vi "Measurement UI.vi"() -> ()   [LabVIEW 2023, in "FPT Intermodulation UI.lvlib"]
uses:
  FPT Intermodulation UI.lvlib
panel:
  in  "Measurement Graph":T1(tab)
  out "Graph Combined":T2(graph)
  out "Graph DUT Gain":T2(graph)
  out "Graph Intermodulation":T2(graph)
  out "Graph TOI":T2(graph)
  out "Graph Fundamental":T2(graph)
  in  "Power sequencing file validity check":bool
  out "TS_Intermodulation Slope (dBm)":dbl[][](array[numeric])
  out "TS_Fundamental Slope (dBm)":dbl[][](array[numeric])
  out "Final Target Pout (dBm)":dbl
  out "All Data":dbl[][](array[numeric])
  out "TS_DUT Gain (dBm)":dbl[][](array[numeric])
  out "TS_TOI (dBm)":dbl[][](array[numeric])
  out "TS_IMD (dBm)":dbl[][](array[numeric])
  out "TS_Fundamental (dBm)":dbl[][](array[numeric])
  out "Typical OIP3 (dBm)":dbl
  out "x-axis label":string
  in  "Power sequencing file path":string
  in  "RFSG name":string="5842_0"
  in  "RFSG attenuation mode":T3(ring)=enum."Constant Attenuation"
  in  "RFSG s2p file path":string
  in  "RFmx name":string="5842_0"
  in  "RFmx attenuation mode":T3(ring)=enum."Constant Attenuation"
  in  "RFmx s2p file path":string
  out "All Graph Reference":refnum<vi>[](array[refnum])
  out "All Plots Data":T4(array[cluster])
  in  "IM_Sweep Mode":enum32{"Power", "Frequency", "Tone Spacing"}(ring) caption="Sweep Mode"
  out "MeasTable_Fix":string[][](table)
  out "MeasTable":string[][](table)
  in  "Tab Control":T5(tab)
  in  "Power sequencing file path_update":path caption="Power Sequencing File Path"
  in  "RFSG name_update":refnum<k15> caption="RFSG Name"
  in  "RFSG attenuation mode_tab":T3(tab)=enum."s2p File" caption="RFSG Attenuation Mode"
  in  "RFSG external attenuation (dB)":dbl caption="External Attenuation" format="%#.3pdB"
  in  "RFSG s2p file path_update":path caption="S2P File Path"
  in  "RFSG s-parameters orientation":enum32{"Port1 Towards DUT", "Port2 Towards DUT"}(ring) caption="Orientation"
  in  "RFmx name_update":refnum<k15> caption="RFmx Name"
  in  "RFmx attenuation mode_tab":T3(tab) caption="RFmx Attenuation Mode"
  in  "RFmx external attenuation (dB)":dbl caption="External Attenuation" format="%#.3pdB"
  in  "RFmx s2p file path_update":path caption="S2P File Path"
  in  "RFmx s-parameters orientation":enum32{"Port1 Towards DUT", "Port2 Towards DUT"}(ring) caption="Orientation"
  in  "RFSG port":string(combo)="port1" caption="RFSG Port"
  in  "RFmx port":string(combo)="port2" caption="RFmx Port"
  in  "RFmx Reference Level (dBm)":dbl=10.0 caption="Reference Level" format="%#.3fdBm"
  in  "RFSG Generation IQ Rate (S/s)":dbl=1250000000.0 caption="Generation IQ Rate" format="%#.3pS/s"
  in  "Start Pin Per Tone (dBm)":dbl=-20.0 caption="Start Pin Per Tone" format="%#.3fdBm"
  in  "Start Center Frequency (Hz)":dbl=8000000000.0 caption="Start Center Frequency" format="%#.3pHz"
  in  "Start Tone Spacing (Hz)":dbl=1000000.0 caption="Start Tone Spacing" format="%#.3pHz"
  in  "Sweep Delay (ms)":u32 format="%#.3pms"
  in  "Sweep Mode_tab":enum32{"Power", "Frequency", "Tone Spacing"}(tab)=enum."Tone Spacing" caption="Sweep Mode"
  in  "Power Sweep End":dbl format="%#.fdBm"
  in  "Power Sweep Step":dbl=1.0 format="%#.fdB"
  in  "Target Pout Per Tone (dBm)":dbl caption="Target Pout Per Tone" format="%#.3fdBm"
  in  "Frequency Sweep End":dbl=12000000000.0 format="%#.pHz"
  in  "Frequency Sweep Step":dbl=100000000.0 format="%#.pHz"
  in  "Tone Spacing Sweep End":dbl=10000000.0 format="%#.pHz"
  in  "Tone Spacing Sweep Step":dbl=1000000.0 format="%#.pHz"
  in  "Mode of operation":T6(ring) caption="Configuration"
  out "Status":string
  # "Intermodulation"
  # "Sweep Options"
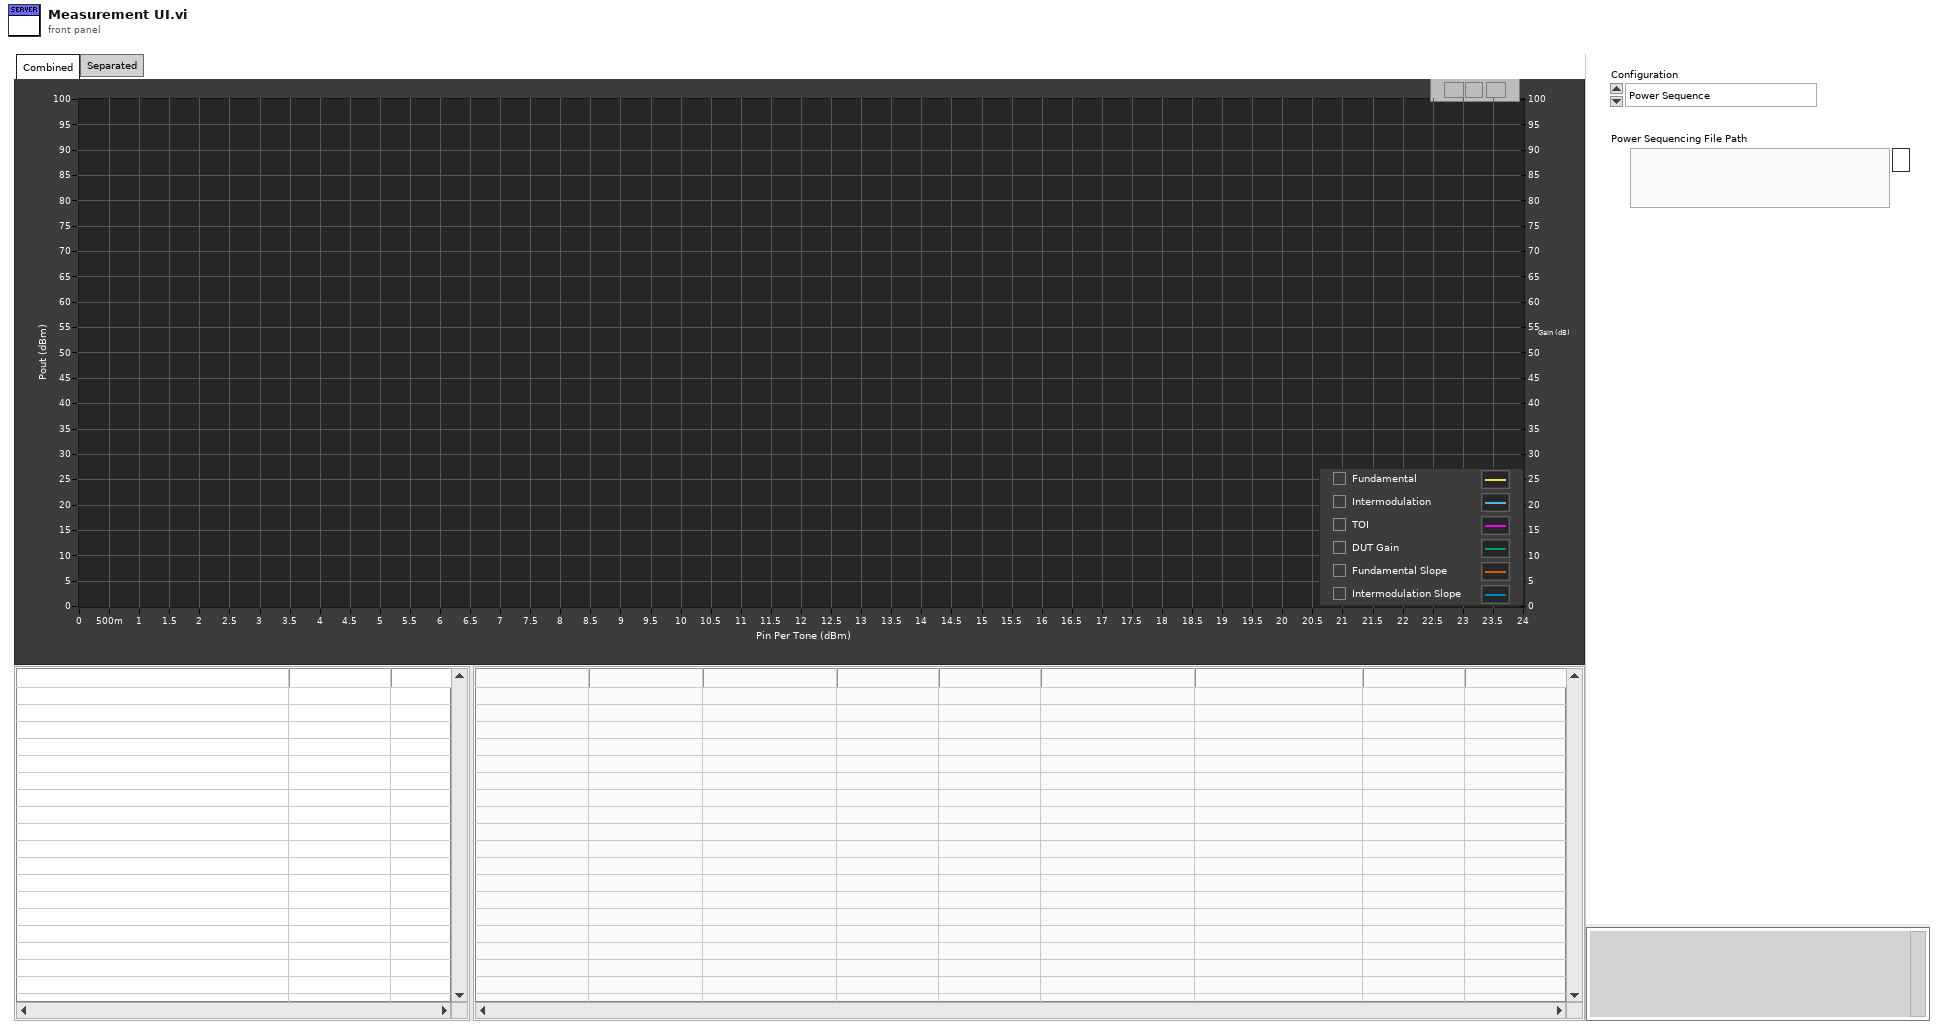
[diagram p1: front panel]
types:
  T1 = enum32{"Combined", "Separated", "Hidden Controls"}
  T2 = cluster{"Load currents":dbl[], "Efficiency":dbl[]}[]
  T3 = enum32{"<None>", "Constant Attenuation", "s2p File"}
  T4 = cluster{"X-axis values":dbl[], "Y-axis values":dbl[]}[]
  T5 = enum32{"Power Sequence", "Correction", "Measurement 1"}
  T6 = enum32{"Power Sequence", "HW + Correction", "Measurement 1"}
  T7 = enum8{"Enabled", "Disabled", "Disabled and Grayed Out"}
  T8 = cluster{"Shift":bool, "Ctrl":bool, "Alt":bool, "Cmd":bool, "Opt":bool}
  T9 = cluster{"TS_Fundamental Slope (dBm)":dbl[], "TS_Fundamental Slope (dBm)":dbl[]}
  T10 = cluster{"TS_Fundamental Slope (dBm)":dbl[], "TS_Intermodulation Slope (dBm)":dbl[]}
  T11 = cluster{"TS_Fundamental Slope (dBm)":dbl[], "TS_Intermodulation Slope (dBm)":dbl[]}[]
  T12 = cluster{"TS_Fundamental (dBm)":dbl[], "TS_Fundamental (dBm)":dbl[]}
  T13 = cluster{"TS_Fundamental (dBm)":dbl[], "TS_IMD (dBm)":dbl[]}
  T14 = cluster{"TS_Fundamental (dBm)":dbl[], "TS_TOI (dBm)":dbl[]}
  T15 = cluster{"TS_Fundamental (dBm)":dbl[], "TS_DUT Gain (dBm)":dbl[]}
  T16 = cluster{"X-axis values":dbl[], "Y-axis values":dbl[]}
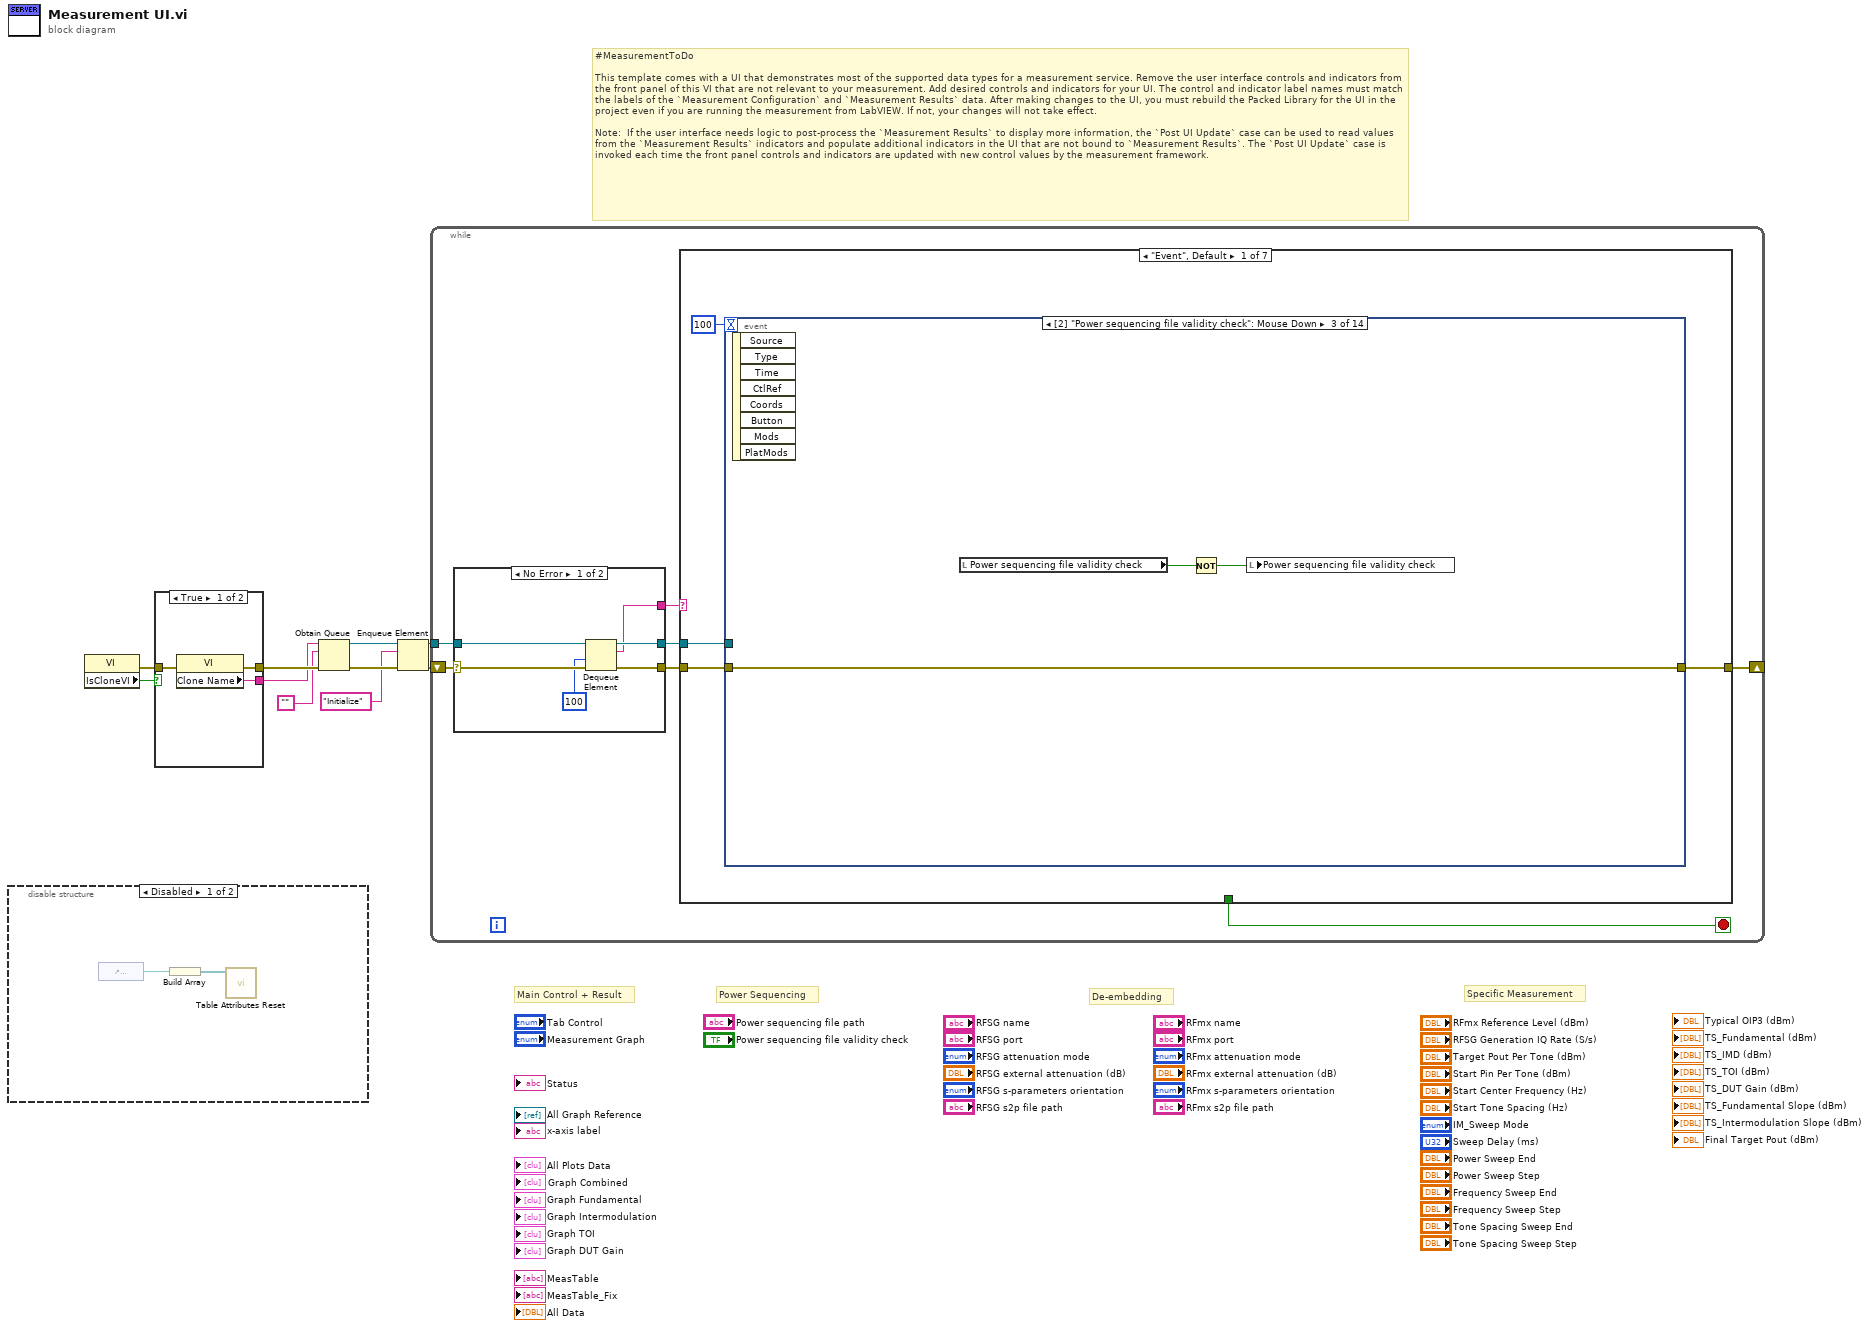
[diagram p0: block diagram]
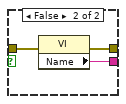
[diagram p3: hidden frame]
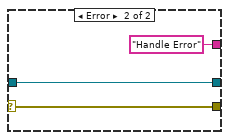
[diagram p4: hidden frame]
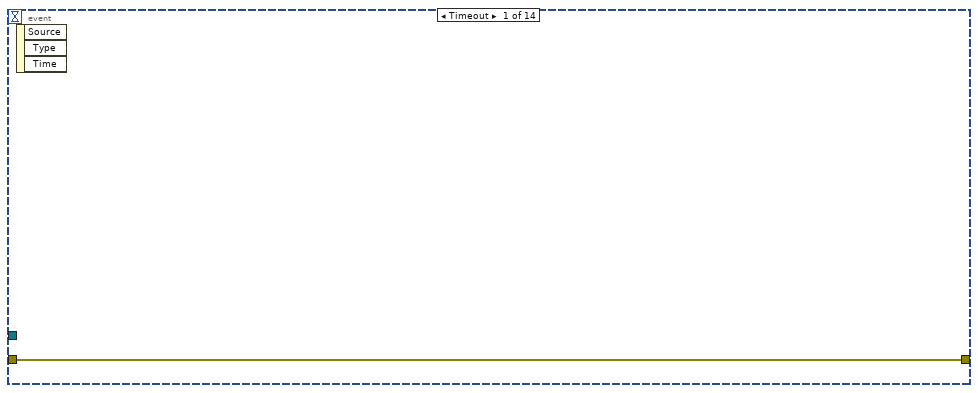
[diagram p5: hidden frame]
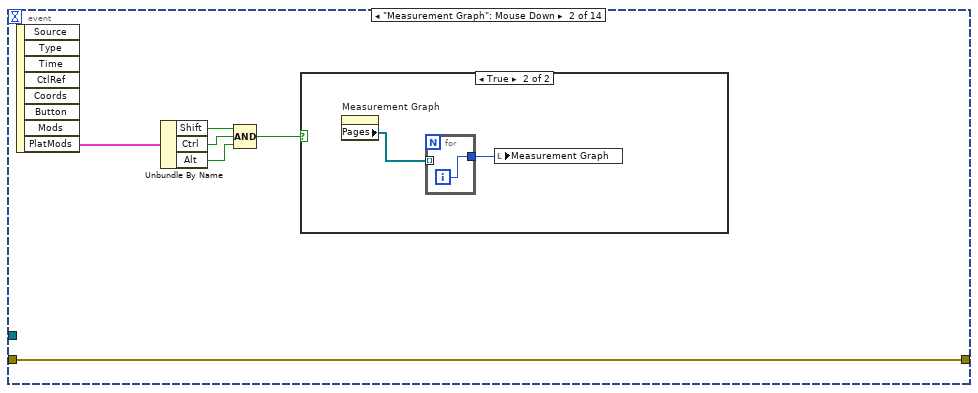
[diagram p6: hidden frame]
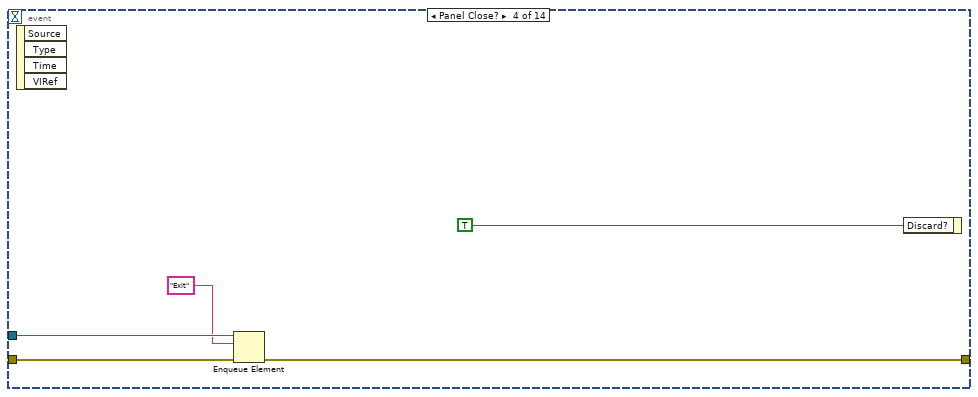
[diagram p8: hidden frame]
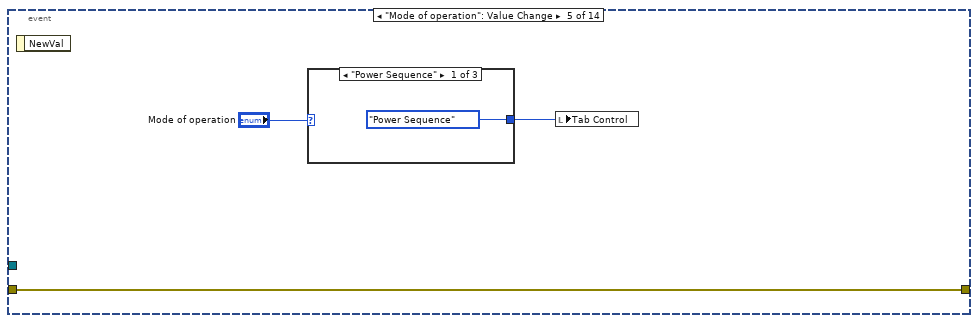
[diagram p9: hidden frame]
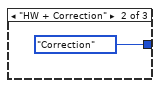
[diagram p10: hidden frame]
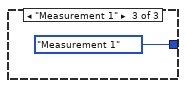
[diagram p11: hidden frame]
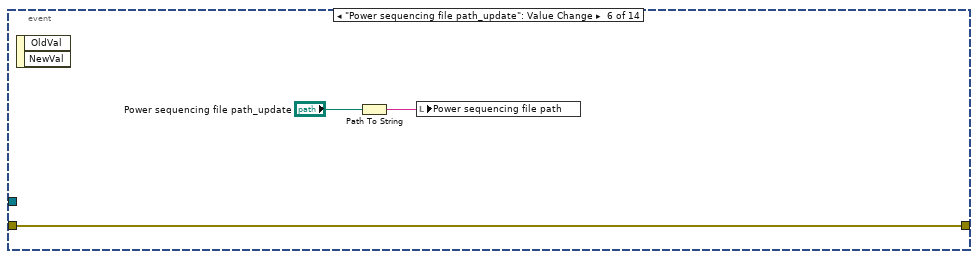
[diagram p12: hidden frame]
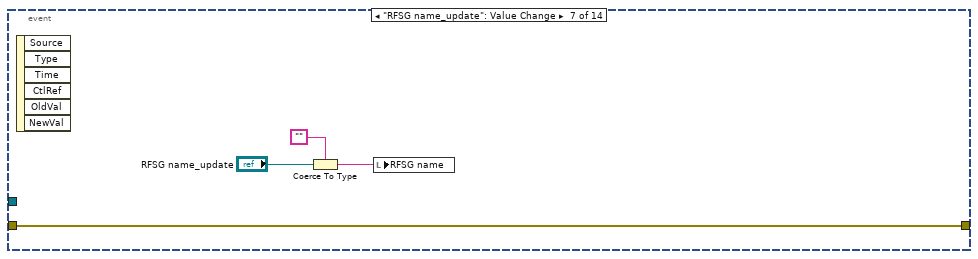
[diagram p13: hidden frame]
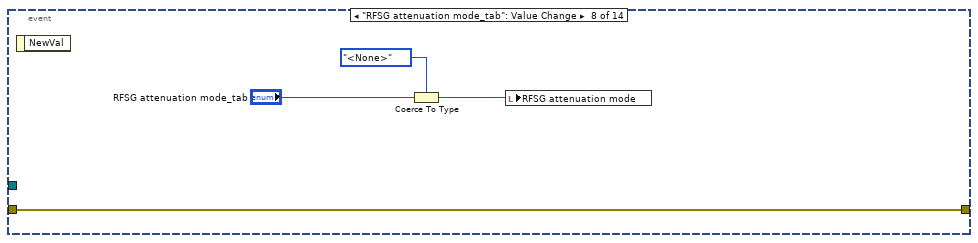
[diagram p14: hidden frame]
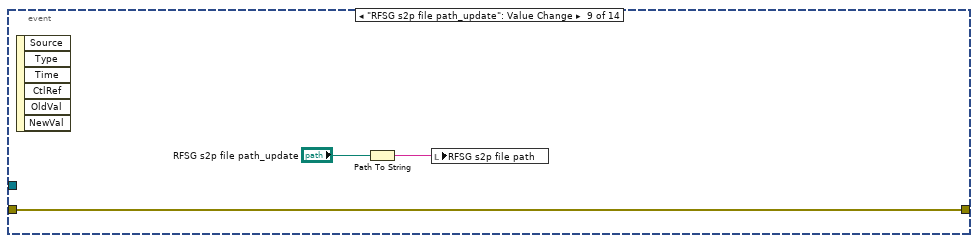
[diagram p15: hidden frame]
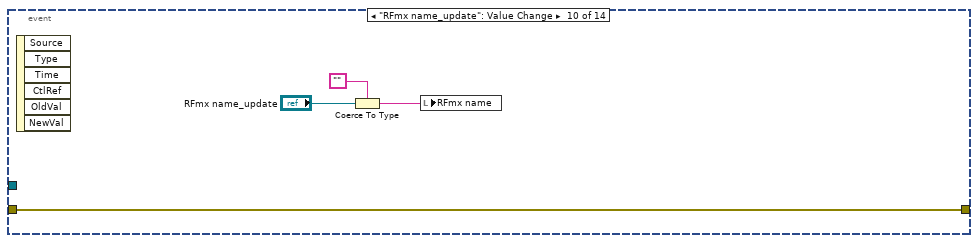
[diagram p16: hidden frame]
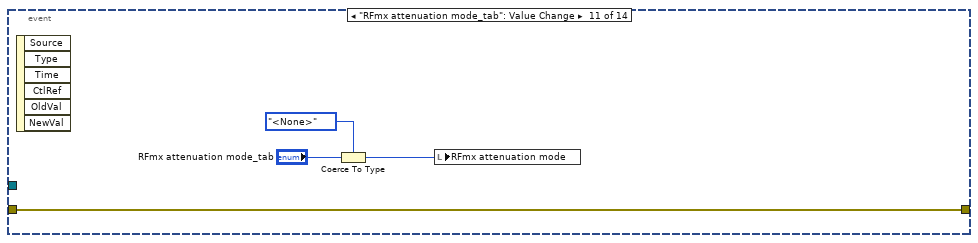
[diagram p17: hidden frame]
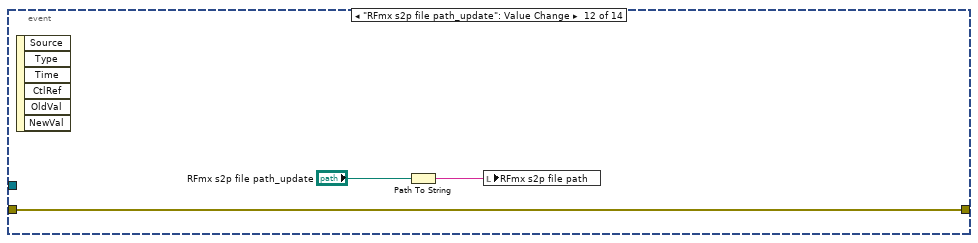
[diagram p18: hidden frame]
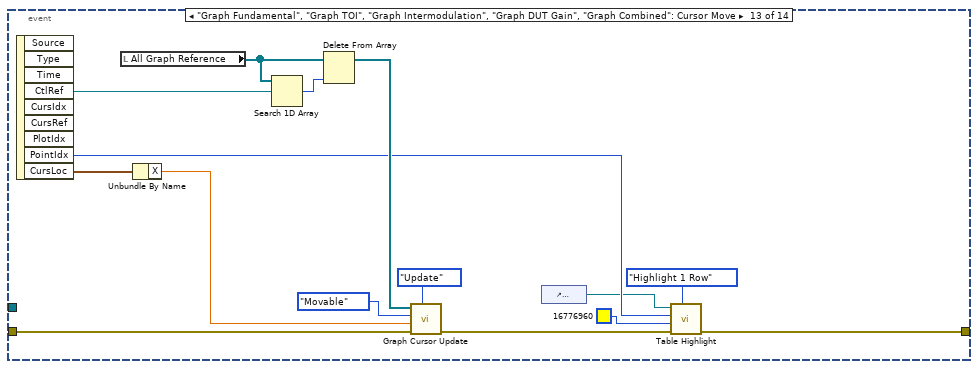
[diagram p19: hidden frame]
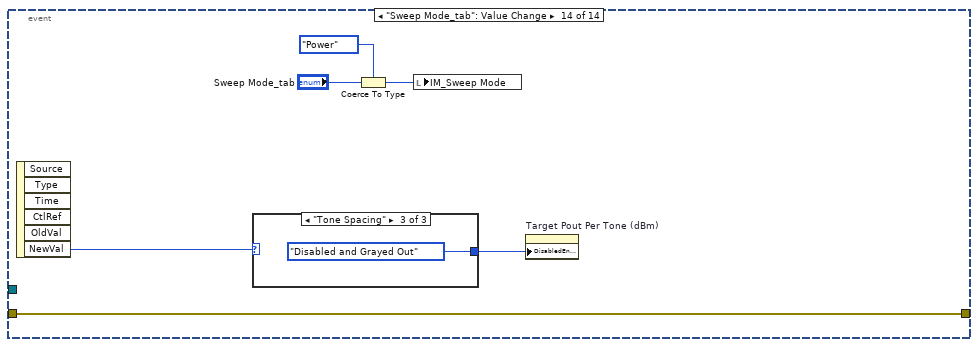
[diagram p20: hidden frame]
diagram:
  # "Specific Measurement"
  # "De-embedding"
  # "Power Sequencing"
  # "Main Control + Result"
  # "#MeasurementToDo  \n\nThis template comes with a UI that demonstrates most of the supported data types for a measurement service. Remove the user interface controls and indicators from the front panel of this VI that are not relevant to your measurement. Add desired controls and indicators for your UI. The control and indicator label names must match the labels of the `Measurement Configuration` and `Measurement Results` data. After making changes to the UI, you must rebuild the Packed Library for the UI in the project even if you are running the measurement from LabVIEW. If not, your changes will not take effect.\n\nNote:  If the user interface needs logic to post-process the `Measurement Results` to display more information, the `Post UI Update` case can be used to read values from the `Measurement Results` indicators and populate additional indicators in the UI that are not bound to `Measurement Results`. The `Post UI Update` case is invoked each time the front panel controls and indicators are updated with new control values by the measurement framework."
  n1 = disable-structure shown="Disabled" {
    frame Disabled {
      n2 = control-ref of="MeasTable"() -> (w12:refnum<vi>)
      n3 = Build Array(w12) -> (w11:refnum<vi>[])
      n4 = call "Table Attributes Reset.vi"("Table Refs"=w11) -> ()  [unwired: 11 in]
    }
    frame Enabled {
    }
  }
  n5 = property class="VI"() -> (error out=w1:errorcluster, "IsCloneVI"=w2:bool)  [unwired: 2 in, 1 out]
  n6 = case shown="True" w2 {
    tunnel: [w15 w18] -> w10
    tunnel: [w14 w17] -> w9
    tunnel: w1 -> [w13 w16]
    frame True {
      n7 = property class="VI"(error in=w13) -> (error out=w15:errorcluster, "Clone Name"=w14:string)  [unwired: 1 in, 1 out]
    }
    frame False {
      n8 = property class="VI"(error in=w16) -> (error out=w18:errorcluster, "Name"=w17:string)  [unwired: 1 in, 1 out]
    }
  }
  n9 = Obtain Queue(name (unnamed)=w9, element data type="", error in (no error)=w10) -> (queue out=w6:refnum<queue>, error out=w8:errorcluster)  [unwired: 2 in, 1 out]
  n10 = Enqueue Element(queue=w6, element="Initialize", error in (no error)=w8) -> (queue out=w5:refnum<queue>, error out=w7:errorcluster)  [unwired: 1 in, 1 out]
  n11 = while {
    shift-right: [w20] -> _
    shift-left: w7 -> [w25]
    tunnel: w5 -> [w23]
    stop <- w19 stop-if-true
    n12 = case shown="No Error" w25 {
      selector: w25 -> [w31 w34]
      tunnel: [w30 w34] -> w24
      tunnel: w23 -> [w29 w33]
      tunnel: [w28 w33] -> w22
      tunnel: [w27 "Handle Error"] -> w21
      frame No Error {
        n13 = Dequeue Element(queue=w29, timeout in ms (-1)=100, error in (no error)=w31) -> (queue out=w28:refnum<queue>, element=w27:string, error out=w30:errorcluster)  [unwired: 1 out]
      }
      frame Error {
      }
    }
    n14 = case shown="\"Event\", Default" w21 {
      tunnel: w24 -> [w37 w123 w175 w216 w240 w254 w255]
      tunnel: w22 -> [w35 _ w174 w215 _ w252 _]
      tunnel: [w38 w123 w175 w205 w240 w249 w255] -> w20
      tunnel: [_ _ _ _ _ TRUE _] -> w19
      frame "Event", Default {
        n15 = event shown="[2] \"Power sequencing file validity check\": Mouse Down" {
          selector: _ -> [_ _ _ _ _ _ _ _ _ _ _ _ _ _]
          dyn-events: _ -> [_ _ _ _ _ _ _ _ _ _ _ _ _ _]
          timeout: 100 -> [_ _ _ _ _ _ _ _ _ _ _ _ _ _]
          tunnel: [w39 w45 w51 w54 w58 w63 w66 w72 w74 w77 w83 w85 w92 w108] -> w38
          tunnel: w37 -> [w39 w45 w51 w55 w58 w63 w66 w72 w74 w77 w83 w85 w102 w108]
          tunnel: w35 -> [_ _ _ w53 _ _ _ _ _ _ _ _ _ _]
          event Timeout {
            n16 = event-data() -> ()  [unwired: 1 in, 3 out]
          }
          event "Measurement Graph": Mouse Down {
            n17 = event-data() -> ("PlatMods"=w44:T8)  [unwired: 1 in, 7 out]
            n18 = Unbundle By Name(w44) -> ("Shift"=w43:bool, "Ctrl"=w42:bool, "Alt"=w41:bool)
            n19 = Compound Arithmetic op=AND(w43, w42, w41) -> (w40:bool)
            n20 = case shown="True" w40 {
              frame False {
              }
              frame True {
                n21 = property on="Measurement Graph" class="TabCtl (strict)"() -> ("Pages"=w47:refnum<vi>[])  [unwired: 2 in, 2 out]
                n22 = for {
                  tunnel: w47 -> [_] mode=indexing
                  tunnel: [w48] -> w46
                  i -> [w48]
                }
                n23 = local write "Measurement Graph"(w46) -> ()
              }
            }
          }
          event "Power sequencing file validity check": Mouse Down {
            n24 = event-data() -> ()  [unwired: 1 in, 8 out]
            n25 = local read "Power sequencing file validity check"() -> (w50:bool)
            n26 = Not(x=w50) -> (.not. x?=w49:bool)
            n27 = local write "Power sequencing file validity check"(w49) -> ()
          }
          event Panel Close? {
            n28 = event-data() -> ()  [unwired: 1 in, 4 out]
            n29 = Enqueue Element(queue=w53, element="Exit", error in (no error)=w55) -> (error out=w54:errorcluster)  [unwired: 1 in, 2 out]
            n30 = event-data("Discard?"=TRUE) -> ()  [unwired: 1 in, 1 out]
          }
          event "Mode of operation": Value Change {
            n31 = event-data() -> ()  [unwired: 1 in, 1 out]
            n32 = case shown="\"Power Sequence\"" "Mode of operation" {
              tunnel: [T5."Power Sequence" ("Tab Control") T5."Correction" ("Tab Control") T5."Measurement 1" ("Tab Control")] -> w57
              frame "Power Sequence" {
              }
              frame "HW + Correction" {
              }
              frame "Measurement 1" {
              }
            }
            n33 = local write "Tab Control"(w57) -> ()
          }
          event "Power sequencing file path_update": Value Change {
            n34 = event-data() -> ()  [unwired: 1 in, 2 out]
            n35 = Path To String(path="Power sequencing file path_update") -> (string=w64:string)
            n36 = local write "Power sequencing file path"(w64) -> ()
          }
          event "RFSG name_update": Value Change {
            n37 = event-data() -> ()  [unwired: 1 in, 6 out]
            n38 = Coerce To Type(0:"RFSG name_update", 1:"") -> (2:w67:string)
            n39 = local write "RFSG name"(w67) -> ()
          }
          event "RFSG attenuation mode_tab": Value Change {
            n40 = event-data() -> ()  [unwired: 1 in, 1 out]
            n41 = Coerce To Type(0:"RFSG attenuation mode_tab", 1:T3."<None>" ("RFSG attenuation mode")) -> (2:w71:T3)
            n42 = local write "RFSG attenuation mode"(w71) -> ()
          }
          event "RFSG s2p file path_update": Value Change {
            n43 = event-data() -> ()  [unwired: 1 in, 6 out]
            n44 = Path To String(path="RFSG s2p file path_update") -> (string=w75:string)
            n45 = local write "RFSG s2p file path"(w75) -> ()
          }
          event "RFmx name_update": Value Change {
            n46 = event-data() -> ()  [unwired: 1 in, 6 out]
            n47 = Coerce To Type(0:"RFmx name_update", 1:"") -> (2:w79:string)
            n48 = local write "RFmx name"(w79) -> ()
          }
          event "RFmx attenuation mode_tab": Value Change {
            n49 = event-data() -> ()  [unwired: 1 in, 6 out]
            n50 = Coerce To Type(0:"RFmx attenuation mode_tab", 1:T3."<None>" ("RFmx attenuation mode")) -> (2:w82:T3)
            n51 = local write "RFmx attenuation mode"(w82) -> ()
          }
          event "RFmx s2p file path_update": Value Change {
            n52 = event-data() -> ()  [unwired: 1 in, 6 out]
            n53 = Path To String(path="RFmx s2p file path_update") -> (string=w86:string)
            n54 = local write "RFmx s2p file path"(w86) -> ()
          }
          event "Graph Fundamental", "Graph TOI", "Graph Intermodulation", "Graph DUT Gain", "Graph Combined": Cursor Move {
            n55 = event-data() -> ("CtlRef"=w100:refnum<vi>, "PointIdx"=w90:i32, "CursLoc"=w101:cluster{"X":dbl, "Y":dbl})  [unwired: 1 in, 6 out]
            n56 = local read "All Graph Reference"() -> (w99:refnum<vi>[])
            n57 = Unbundle By Name(w101) -> ("X"=w95:dbl)
            n58 = Search 1D Array(1D array=w99, element=w100) -> (index of element=w98:i32)  [unwired: 1 in]
            n59 = Delete From Array(array=w99, index=w98) -> (array with subset deleted=w97:refnum<vi>[])  [unwired: 1 in, 1 out]
            n60 = call "Graph Cursor Update.vi"("Action"=enum16{"Reset", "Update"}."Update", "error in"=w102, "New X position"=w95, "Cursor Type"=enum16{"Movable", "Fixed", "All"}."Movable", "Graph Refs in"=w97) -> ("error out"=w93:errorcluster)  [unwired: 5 in, 1 out]
            n61 = control-ref of="MeasTable"() -> (w89:refnum<vi>)
            n62 = call "Table Highlight.vi"("Action"=enum16{"Reset", "Highlight 1 Row"}."Highlight 1 Row", "error in"=w93, "Color Box"=u32 16776960, "Row"=w90, "Table Ref in"=w89) -> ("error out"=w92:errorcluster)  [unwired: 5 in, 1 out]
          }
          event "Sweep Mode_tab": Value Change {
            n63 = event-data() -> ("NewVal"=w103:enum32{"Power", "Frequency", "Tone Spacing"})  [unwired: 1 in, 5 out]
            n64 = case shown="\"Tone Spacing\"" w103 {
              tunnel: [T7."Disabled and Grayed Out" ("Disabled") T7."Enabled" ("Disabled") T7."Disabled and Grayed Out" ("Disabled")] -> w104
              frame "Frequency" {
              }
              frame "Power" {
              }
              frame "Tone Spacing" {
              }
            }
            n65 = Coerce To Type(0:"Sweep Mode_tab", 1:enum32{"Power", "Frequency", "Tone Spacing"}."Power" ("IM_Sweep Mode")) -> (2:w105:enum32{"Power", "Frequency", "Tone Spacing"})
            n66 = local write "IM_Sweep Mode"(w105) -> ()
            n67 = property on="Target Pout Per Tone (dBm)" class="DigNum (strict)"("DisabledEnum"=w104) -> ()  [unwired: 2 in, 2 out]
          }
        }
      }
      frame "Initialize" {
        w118 = 0
        n68 = local write "Tab Control"(w118) -> ()
        n69 = local write "Mode of operation"(w118) -> ()
        n70 = control-ref of="Graph Combined"() -> (w117:refnum<vi>)
        n71 = control-ref of="Graph Fundamental"() -> (w122:refnum<vi>)
        n72 = control-ref of="Graph Intermodulation"() -> (w120:refnum<vi>)
        n73 = control-ref of="Graph TOI"() -> (w119:refnum<vi>)
        n74 = control-ref of="Graph DUT Gain"() -> (w121:refnum<vi>)
        n75 = Build Array(w117, w122, w120, w119, w121) -> (w116:refnum<vi>[])
        n76 = property on="All Graph Reference" class="Arr (strict)"("Value"=w116) -> ()  [unwired: 2 in, 2 out]
        n77 = call "Graph Set Cursor Mode.vi"("Cursor Mode"=enum32{"Free-Drag", "Single-Plot", "Multi-Plot"}."Multi-Plot", "Graph Refs in"=w116) -> ("Graph Refs out"=w114:refnum<vi>[])  [unwired: 8 in, 1 out]
        n78 = call "Graph Cursor Update.vi"("Action"=enum16{"Reset", "Update"}."Reset", "Cursor Type"=enum16{"Movable", "Fixed", "All"}."All", "Graph Refs in"=w114) -> ()  [unwired: 7 in, 2 out]
      }
      frame "Post UI Update" {
        # "This case will be triggered, after framework updates the User interface with result values.\nUsed to update data type def and store data"
        n79 = local read "Power sequencing file path"() -> (w171:string)
        n80 = local read "RFSG name"() -> (w169:string)
        n81 = local read "RFSG attenuation mode"() -> (w170:T3)
        n82 = local read "RFSG s2p file path"() -> (w165:string)
        n83 = local read "TS_Fundamental (dBm)"() -> (w125:dbl[][])
        n84 = local read "TS_DUT Gain (dBm)"() -> (w152:dbl[][])
        n85 = local read "TS_IMD (dBm)"() -> (w154:dbl[][])
        n86 = local read "TS_TOI (dBm)"() -> (w153:dbl[][])
        n87 = Enqueue Element(queue=w174, element="Post UI Update 2") -> ()  [unwired: 2 in, 3 out]
        n88 = Coerce To Type(0:w169, 1:refnum<k15> refnum ("RFSG name_update")) -> (2:w167:refnum<k15>)
        n89 = String To Path(string=w165) -> (path=w166:path)
        n90 = local read "IM_Sweep Mode"() -> (w126:enum32{"Power", "Frequency", "Tone Spacing"})
        n91 = local write "RFSG name_update"(w167) -> ()
        n92 = Coerce To Type(0:w170, 1:T3."<None>" ("RFSG attenuation mode_tab")) -> (2:w158:T3)
        n93 = local write "RFSG s2p file path_update"(w166) -> ()
        n94 = Index Array(array=w125) -> (element #1=w133:dbl[], element #2=w124:dbl[])  [unwired: 4 in]
        n95 = Index Array(array=w154, index (row)=1) -> (element=w141:dbl[])  [unwired: 1 in]
        n96 = Index Array(array=w153, index (row)=1) -> (element=w139:dbl[])  [unwired: 1 in]
        n97 = Index Array(array=w152, index (row)=1) -> (element=w136:dbl[])  [unwired: 1 in]
        n98 = String To Path(string=w171) -> (path=w172:path)
        n99 = local write "RFSG attenuation mode_tab"(w158) -> ()
        n100 = local write "Power sequencing file path_update"(w172) -> ()
        n101 = case shown="\"Power\", Default" w126 {
          tunnel: [w183 _ _] -> w135
          tunnel: [w180 _ _] -> w144
          tunnel: w133 -> [_ w186 w188]
          tunnel: [w182 _ _] -> w134
          tunnel: ["Pin Per Tone (dBm)" "Frequency (GHz)" "Tone Spacing (MHz)"] -> w151
          tunnel: [w177 w186 w188] -> w137
          frame "Power", Default {
            n102 = local read "TS_Intermodulation Slope (dBm)"() -> (w184:dbl[][])
            n103 = local read "TS_Fundamental Slope (dBm)"() -> (w185:dbl[][])
            n104 = local read "Final Target Pout (dBm)"() -> (w176:dbl)
            n105 = local write "Target Pout Per Tone (dBm)"(w176) -> ()
            n106 = Index Array(array=w185) -> (element #1=w177:dbl[], element #2=w183:dbl[])  [unwired: 4 in]
            n107 = Index Array(array=w184) -> (element #2=w182:dbl[])  [unwired: 4 in, 1 out]
            n108 = Bundle("TS_Fundamental Slope (dBm)"=w177, "TS_Fundamental Slope (dBm)"=w183) -> (w181:T9)  [unwired: 1 in]
            n109 = Bundle("TS_Fundamental Slope (dBm)"=w177, "TS_Intermodulation Slope (dBm)"=w182) -> (w179:T10)  [unwired: 1 in]
            n110 = Build Array(w181, w179) -> (w180:T11)
          }
          frame "Frequency" {
          }
          frame "Tone Spacing" {
          }
        }
        n111 = local read "RFmx name"() -> (w160:string)
        n112 = local read "RFmx attenuation mode"() -> (w159:T3)
        n113 = local read "RFmx s2p file path"() -> (w164:string)
        n114 = local read "IM_Sweep Mode"() -> (w132:enum32{"Power", "Frequency", "Tone Spacing"})
        n115 = Coerce To Type(0:w160, 1:refnum<k15> refnum ("RFSG name_update")) -> (2:w162:refnum<k15>)
        n116 = local write "RFmx name_update"(w162) -> ()
        n117 = Coerce To Type(0:w132, 1:enum32{"Power", "Frequency", "Tone Spacing"}."Power" ("Sweep Mode_tab")) -> (2:w130:enum32{"Power", "Frequency", "Tone Spacing"})
        n118 = String To Path(string=w164) -> (path=w163:path)
        n119 = Coerce To Type(0:w159, 1:T3."<None>" ("RFmx attenuation mode_tab")) -> (2:w156:T3)
        n120 = call "Resize Data with xi-axis (NaN).vi"("x-axis"=w137, "Measure data"=w124) -> ("Updated Data"=w143:dbl[])  [unwired: 13 in]
        n121 = call "Resize Data with xi-axis (NaN).vi"("x-axis"=w137, "Measure data"=w141) -> ("Updated Data"=w142:dbl[])  [unwired: 13 in]
        n122 = call "Resize Data with xi-axis (NaN).vi"("x-axis"=w137, "Measure data"=w139) -> ("Updated Data"=w140:dbl[])  [unwired: 13 in]
        n123 = call "Resize Data with xi-axis (NaN).vi"("x-axis"=w137, "Measure data"=w136) -> ("Updated Data"=w138:dbl[])  [unwired: 13 in]
        n124 = local write "Sweep Mode_tab"(w130) -> ()
        n125 = Bundle("TS_Fundamental (dBm)"=w137, "TS_Fundamental (dBm)"=w124) -> (w148:T12)  [unwired: 1 in]
        n126 = Bundle("TS_Fundamental (dBm)"=w137, "TS_IMD (dBm)"=w141) -> (w147:T13)  [unwired: 1 in]
        n127 = Bundle("TS_Fundamental (dBm)"=w137, "TS_TOI (dBm)"=w139) -> (w146:T14)  [unwired: 1 in]
        n128 = Bundle("TS_Fundamental (dBm)"=w137, "TS_DUT Gain (dBm)"=w136) -> (w145:T15)  [unwired: 1 in]
        n129 = local write "RFmx attenuation mode_tab"(w156) -> ()
        n130 = local write "RFmx s2p file path_update"(w163) -> ()
        n131 = Build Array(w137, w143, w142, w140, w138, w135, w134) -> (w150:dbl[][])
        n132 = Build Array (concatenate)(w148, w147, w146, w145, w144) -> (w149:T11)
        n133 = property on="x-axis label" class="Str"("Value"=w151) -> ()  [unwired: 2 in, 2 out]
        n134 = local write "All Plots Data"(w149) -> ()
        n135 = local write "All Data"(w150) -> ()
      }
      frame "Post UI Update 2" {
        # "#ToBeImprove\n- highlight or bold the row with expected Pout\n- hide the cursor when not using power sweep"
        # "update Target Pout Per Tone"
        # "Run after Post UI Update. Can be duplicate is need more processing.\nUpdate all data to graph"
        n136 = Enqueue Element(queue=w215, element="Post UI Update 3", error in (no error)=w216) -> (error out=w193:errorcluster)  [unwired: 1 in, 2 out]
        n137 = local read "All Graph Reference"() -> (w191:refnum<vi>[])
        n138 = local read "All Plots Data"() -> (w201:T4)
        n139 = local read "x-axis label"() -> (w190:string)
        n140 = control-ref of="Graph Combined"() -> (w204:refnum<vi>)
        n141 = Build Array(w204) -> (w203:refnum<vi>[])
        n142 = for {
          tunnel: w191 -> [w219] mode=indexing
          shift-right: [w220] -> w192
          shift-left: w193 -> [w221]
          tunnel: w190 -> [w218]
          n143 = property class="XYGraph (strict)"(reference=w219, error in=w221, "XScale.NameLbl.Text"=w218) -> (error out=w220:errorcluster)  [unwired: 1 out]
        }
        n144 = call "Graph Update.vi"("Graph Type"=enum16{"Combined", "Multiple"}."Combined", "Graph Plots"=w201, "Graph Reference in"=w203) -> ()  [unwired: 8 in, 1 out]
        n145 = local read "Target Pout Per Tone (dBm)"() -> (w213:dbl)
        n146 = local read "All Plots Data"() -> (w212:T4)
        n147 = local read "x-axis label"() -> (w214:string)
        n148 = control-ref of="Graph Fundamental"() -> (w200:refnum<vi>)
        n149 = control-ref of="Graph Intermodulation"() -> (w199:refnum<vi>)
        n150 = control-ref of="Graph TOI"() -> (w198:refnum<vi>)
        n151 = control-ref of="Graph DUT Gain"() -> (w197:refnum<vi>)
        n152 = Index Array(array=w212) -> (element=w211:T16)  [unwired: 1 in]
        n153 = local read "All Plots Data"() -> (w194:T4)
        n154 = call "Get Pin at Target Pout.vi"("error in"=w192, "x-axis name"=w214, "IM_Target Pout Per Tone (dBm)"=w213, "Graph Data"=w211) -> ("error out"=w210:errorcluster, "Pin @ Target Pout"=w206:dbl)  [unwired: 6 in]
        n155 = Build Array(w200, w199, w198, w197) -> (w196:refnum<vi>[])
        n156 = local read "All Graph Reference"() -> (w208:refnum<vi>[])
        n157 = call "Graph Update.vi"("Graph Type"=enum16{"Combined", "Multiple"}."Multiple", "Graph Plots"=w194, "Graph Reference in"=w196) -> ()  [unwired: 8 in, 1 out]
        n158 = call "Graph Cursor Update.vi"("Action"=enum16{"Reset", "Update"}."Update", "error in"=w210, "New X position"=w206, "Cursor Type"=enum16{"Movable", "Fixed", "All"}."Fixed", "Graph Refs in"=w208) -> ("error out"=w205:errorcluster)  [unwired: 5 in, 1 out]
      }
      frame "Post UI Update 3" {
        # "Run after Post UI Update. Can be duplicate is need more processing.\nUpdate data into table"
        n159 = local read "x-axis label"() -> (w236:string)
        n160 = Equal?(x=w236, y="Pin Per Tone (dBm)") -> (x = y?=w226:bool)
        n161 = case shown="True" w226 {
          tunnel: [w242 string[] ["Fundamental Slope (dBm)", "Intermodulation Slope (dBm)"]] -> w225
          tunnel: [2 ("length") 0 ("length")] -> w222
          frame False {
            n162 = Build Array("") -> (w242:string[])
          }
          frame True {
          }
        }
        n163 = case shown="False" w226 {
          tunnel: [string[] ["Output Third-Order Intercept (OIP3)"] string[] ["Typical Output Third-Order Intercept (OIP3)"]] -> w235
          frame True {
          }
          frame False {
          }
        }
        n164 = local read "x-axis label"() -> (w229:string)
        n165 = local read "Typical OIP3 (dBm)"() -> (w234:dbl)
        n166 = Build Array (concatenate)(w229, string[] ["Fundamental (dBm)", "Intermodulation (dBm)", "TOI (dBm)", "DUT Gain (dBm)"], w225) -> (w227:string[])
        n167 = local read "All Data"() -> (w224:dbl[][])
        n168 = Build Array(w234) -> (w233:dbl[])
        n169 = control-ref of="MeasTable_Fix"() -> (w238:refnum<vi>)
        n170 = control-ref of="MeasTable"() -> (w239:refnum<vi>)
        n171 = Build Array(w233) -> (w232:dbl[][])
        n172 = Delete From Array(array=w224, length=w222) -> (array with subset deleted=w223:dbl[][])  [unwired: 2 in, 1 out]
        n173 = call "Table Set Header Name and Data (DBL).vi"("format string"="%#.3p" ("Results Num Format"), "Data"=w232, "Header"=w235, "Table Ref"=w238) -> ()  [unwired: 8 in]
        n174 = call "Table Set Header Name and Data (DBL).vi"("format string"="%#.3p" ("Results Num Format"), "Data"=w223, "Header"=w227, "Table Ref"=w239) -> ()  [unwired: 8 in]
      }
      frame "Exit" {
        # "This case is triggered to close the User Interface from framework"
        n175 = Flush Queue(queue=w252, error in (no error)=w254) -> (queue out=w251:refnum<queue>, error out=w250:errorcluster)  [unwired: 1 out]
        n176 = Release Queue(queue=w251, force destroy? (F)=TRUE, error in (no error)=w250) -> (error out=w249:errorcluster)  [unwired: 2 out]
      }
      frame "Handle Error" {
      }
    }
  }
